vi "VIH Utility - UI - Boolean to Control Disable Status.vi"(0 "Status in":bool) -> (2 "Control Disable if True":u8, 3 "Control Disable if False":u8)   [LabVIEW 2014]
doc: "::: VI Helpeks :::\nCopyright (c) 2000-2026 Konstantin Shifershteyn. All rights reserved."
panel:
  # "VI Helpeks\nCopyright (c) 2012-2026 Konstantin Shifershteyn"
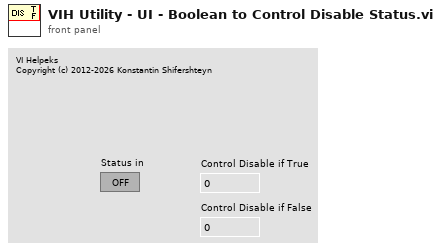
[diagram p1: front panel]
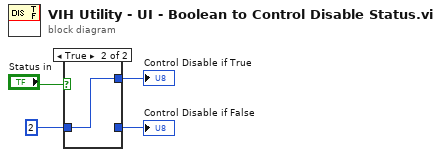
[diagram p0: block diagram]
diagram:
  n1 = case shown="True" "Status in" {
    tunnel: [_ w6] -> w3
    tunnel: u8 2 ("Control Disable if False") -> [w5 w6]
    tunnel: [w5 _] -> w1
    frame False {
    }
    frame True {
    }
  }
  "Control Disable if True" <- w3
  "Control Disable if False" <- w1
